vi "New root not relative--error.vi"() -> (0 "error out":errorcluster)   [LabVIEW 2026]
doc: "The provided new root folder does not lie inside the current root."
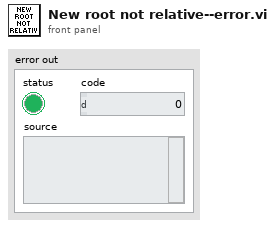
[diagram p1: front panel]
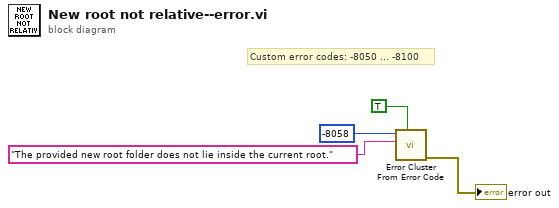
[diagram p0: block diagram]
diagram:
  # "Custom error codes: -8050 ... -8100"
  n1 = call <vilib>:"Error Cluster From Error Code.vi"("show call chain? (False)"=TRUE, "error message (\"\")"="The provided new root folder does not lie inside the current root." ("error message (\"\")"), "error code (0)"=-8058) -> ("error out"=→"error out":errorcluster)  [unwired: 6 in]
